vi "Update U8 Monitor DVR.vi"(8 "error in (no error)":errorcluster, 10 "pcap CAN Data in":u8[](array[numeric]), 11 "CAN_Reader_NIXNET_Plugin in":refnum<class "CAN_Reader_CANsub_Plugin.lvclass">) -> (0 "error out":errorcluster, 2 "pcap CAN Data out":u8[](array[numeric]), 3 "CAN_Reader_NIXNET_Plugin out":refnum<class "CAN_Reader_CANsub_Plugin.lvclass">)   [LabVIEW 2021, in "CAN_Reader_CANsub_Plugin.lvclass"]
uses:
  CAN_Reader_CANsub_Plugin.lvclass
  CAN_Reader_CANsub_Plugin.lvclass/CAN_Reader_CANsub_Plugin.ctl
  <vilib>/CIF Foundation/CIF U8 Array Monitor gRPC/U8_Array_Monitor_gRPC/CIFU8ArrayMonitorUtilities/CIFU8ArrayMonitorUtilities.lvlib
  <vilib>/CIF Foundation/CIF U8 Array Monitor gRPC/U8_Array_Monitor_gRPC/CIFU8ArrayMonitorUtilities/Typedef/U8 Array.ctl
  <vilib>/CIF Foundation/CIF Utilities/Time/Time_CIF_U.lvlib
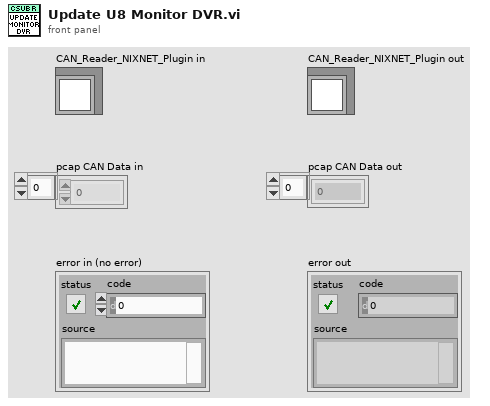
[diagram p1: front panel]
types:
  T1 = typedef "U8 Array.ctl" = cluster{"Timestamp":i64, "U8 Array":u8[]}
  T2 = typedef "CIFU8ArrayMonitorUtilities.lvlib/CIF U8 Array DVR.ctl" = refnum<data-value>
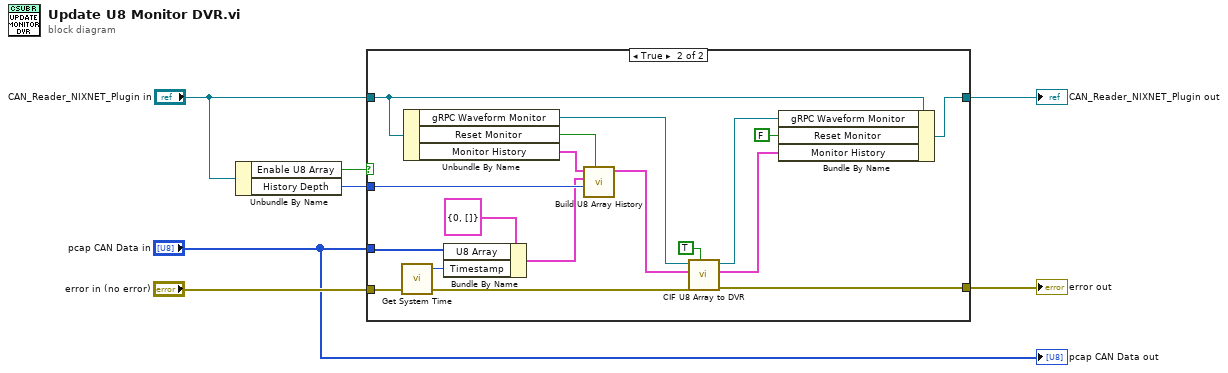
[diagram p0: block diagram]
diagram:
  n1 = Unbundle By Name("CAN_Reader_NIXNET_Plugin in") -> ("Enable U8 Array"=w5:bool, "History Depth"=w2:u32)
  n2 = case shown="True" w5 {
    tunnel: "error in (no error)" -> [w8 w26]
    tunnel: [w8 w25] -> w6
    tunnel: "CAN_Reader_NIXNET_Plugin in" -> [w9 w21]
    tunnel: [w9 w15] -> w3
    tunnel: w2 -> [_ w24]
    tunnel: "pcap CAN Data in" -> [_ w14]
    frame False {
    }
    frame True {
      n3 = call <vilib>:"Get System Time.vi"() -> ("Time (ns)"=w12:i64)  [unwired: 5 in]
      n4 = Unbundle By Name(w21) -> ("gRPC Waveform Monitor"=w19:T2, "Reset Monitor"=w22:bool, "Monitor History"=w23:T1[])
      n5 = Bundle By Name(cluster=T1 {"Timestamp"=0, "U8 Array"=[]} ("U8 Array Data"), "U8 Array"=w14, "Timestamp"=w12) -> (w11:T1)
      n6 = call <vilib>:"Build U8 Array History.vi"("Reset"=w22, "History depth"=w24, "U8 Array Data"=w11, "CIF U8 History in"=w23) -> ("CIF U8 History out"=w20:T1[])  [unwired: 7 in]
      n7 = call <vilib>:"CIF U8 Array to DVR.vi"("gRPC U8 Array Enabled"=TRUE, "error in (no error)"=w26, "CIF U8 Array in"=w20, "gRPC U8 Array Monitor in"=w19) -> ("error out"=w25:errorcluster, "CIF U8 Array out"=w18:T1[], "gRPC U8 Array Monitor out"=w17:T2)  [unwired: 5 in]
      n8 = Bundle By Name(cluster=w21, "gRPC Waveform Monitor"=w17, "Reset Monitor"=FALSE, "Monitor History"=w18) -> (w15:refnum<class "CAN_Reader_CANsub_Plugin.lvclass">)
    }
  }
  "error out" <- w6
  "CAN_Reader_NIXNET_Plugin out" <- w3
  "pcap CAN Data out" <- "pcap CAN Data in"
